vi "Create Value - Known Type.vi"(5 "JSON Compatible Type":T1=enum."Unknown", 7 "JSON Type":T2=enum."Unknown", 8 "error in (no error)":errorcluster, 10 "Value":variant) -> (0 "error out":errorcluster, 3 "JSON Tree":variant)   [LabVIEW 2014, in "i3-json.lvlib"]
doc: "Creates a new JSON Object of the given type"
uses:
  i3-json.lvlib
  JSON Types/JSON Type.ctl
  JSON Types/JSON Compatible Type.ctl
  JSON Types/JSON Variant Attribute.ctl
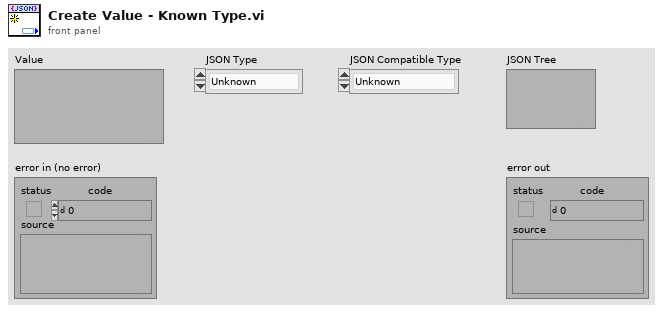
[diagram p1: front panel]
types:
  T1 = typedef "i3-json.lvlib/JSON Compatible Type.ctl" = enum16{"1D Double Array", "1D String Array", "1D Boolean Array", "Unknown"}
  T2 = typedef "i3-json.lvlib/JSON Type.ctl" = enum8{"JSON Compatible", "JSON Array", "JSON Object", "JSON Null", "Double", "String", "Boolean", "Unknown"}
  T3 = typedef "i3-json.lvlib/JSON Variant Attribute.ctl" = string
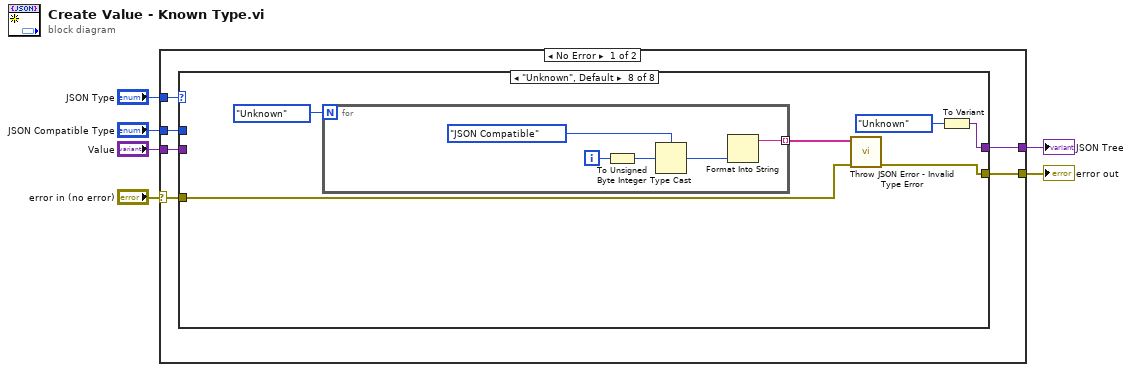
[diagram p0: block diagram]
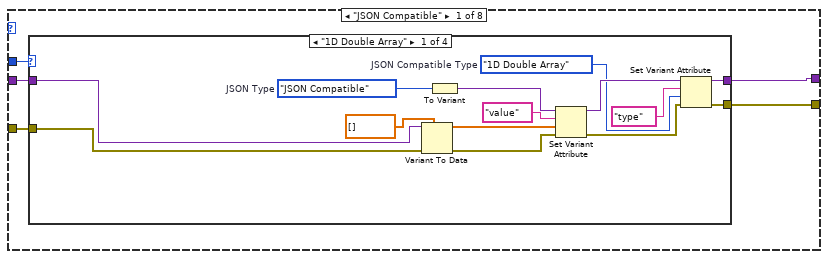
[diagram p2: hidden frame]
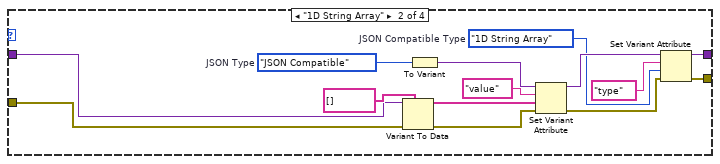
[diagram p3: hidden frame]
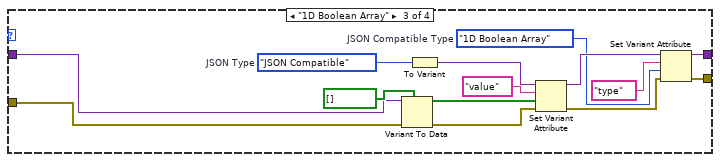
[diagram p4: hidden frame]
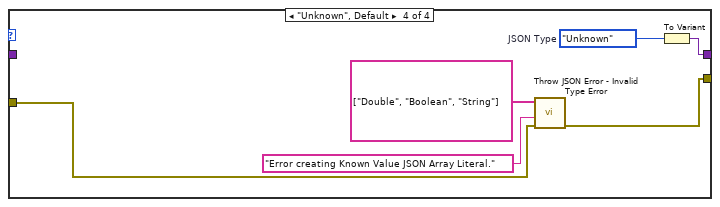
[diagram p5: hidden frame]
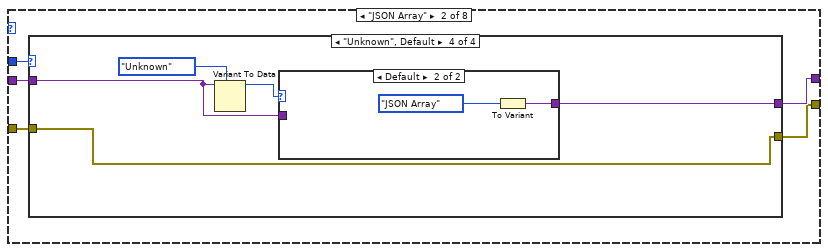
[diagram p6: hidden frame]
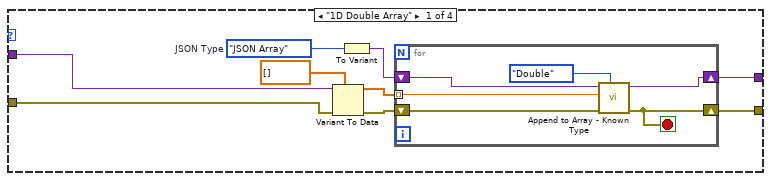
[diagram p7: hidden frame]
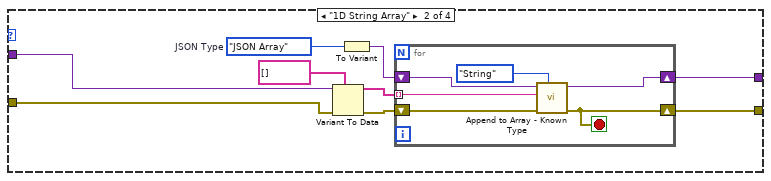
[diagram p8: hidden frame]
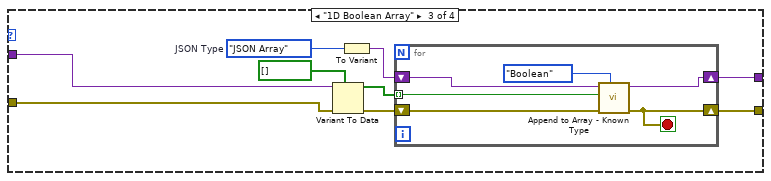
[diagram p9: hidden frame]
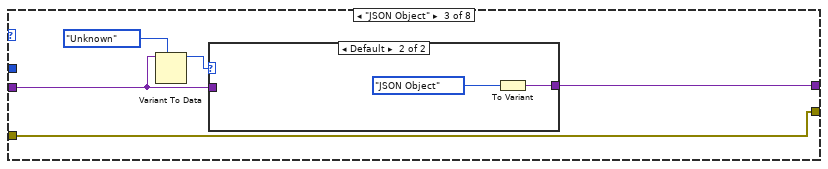
[diagram p11: hidden frame]
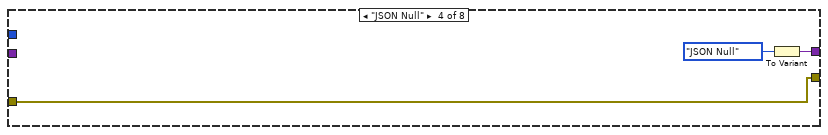
[diagram p13: hidden frame]
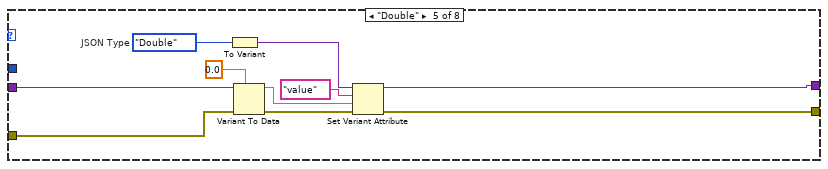
[diagram p14: hidden frame]
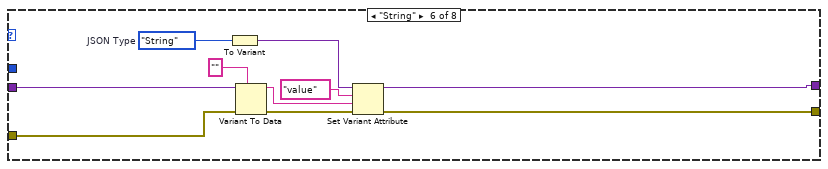
[diagram p15: hidden frame]
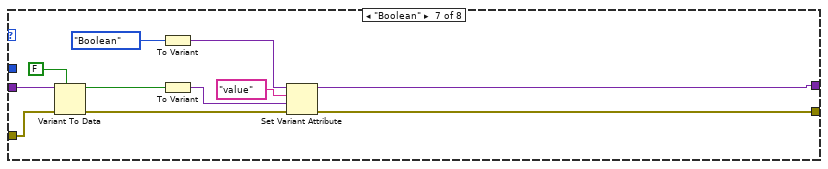
[diagram p16: hidden frame]
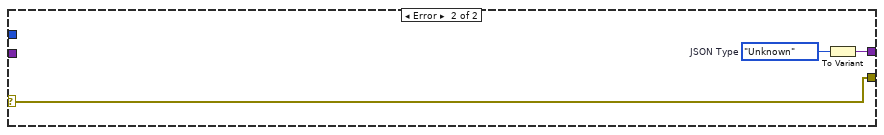
[diagram p17: hidden frame]
diagram:
  n1 = case shown="No Error" "error in (no error)" {
    selector: "error in (no error)" -> [w11 w177]
    tunnel: [w12 w177] -> w5
    tunnel: [w10 w178] -> w4
    tunnel: "JSON Type" -> [w9 _]
    tunnel: "JSON Compatible Type" -> [w8 _]
    tunnel: "Value" -> [w7 _]
    frame No Error {
      n2 = case shown="\"Unknown\", Default" w9 {
        tunnel: [w15 w66 w128 w132 w137 w147 w156 w168] -> w12
        tunnel: w11 -> [w14 w69 w128 w132 w143 w153 w163 w169]
        tunnel: [w16 w70 w125 w133 w135 w148 w157 w171] -> w10
        tunnel: w7 -> [w13 w67 w126 _ w142 w152 w164 _]
        tunnel: w8 -> [w17 w68 _ _ _ _ _ _]
        frame "JSON Compatible" {
          n3 = case shown="\"1D Double Array\"" w17 {
            tunnel: [w19 w38 w53 w64] -> w16
            tunnel: [w18 w37 w52 w60] -> w15
            tunnel: w14 -> [w22 w32 w47 w61]
            tunnel: w13 -> [w21 w35 w46 _]
            frame "1D Double Array" {
              w25 = JSON_Compatible_Type."1D Double Array"  # JSON Compatible Type
              w31 = JSON_Type."JSON Compatible"  # JSON Type
              n4 = Variant To Data(error in=w22, type=dbl[] [], Variant=w21) -> (data=w20:dbl[], error out=w23:errorcluster)
              n5 = To Variant(anything=w31) -> (Variant=w30:variant)
              n6 = Set Variant Attribute(Variant=w30, name=T3 "value" ("JSON Variant Attribute"), value=w20, error in=w23) -> (Variant out=w27:variant, error out=w29:errorcluster)  [unwired: 1 out]
              n7 = Set Variant Attribute(Variant=w27, name=T3 "type" ("JSON Variant Attribute"), value=w25, error in=w29) -> (Variant out=w19:variant, error out=w18:errorcluster)  [unwired: 1 out]
            }
            frame "1D String Array" {
              w39 = JSON_Compatible_Type."1D String Array"  # JSON Compatible Type
              w45 = JSON_Type."JSON Compatible"  # JSON Type
              n8 = Variant To Data(error in=w32, type=string[] [], Variant=w35) -> (data=w34:string[], error out=w33:errorcluster)
              n9 = To Variant(anything=w45) -> (Variant=w44:variant)
              n10 = Set Variant Attribute(Variant=w44, name=T3 "value" ("JSON Variant Attribute"), value=w34, error in=w33) -> (Variant out=w41:variant, error out=w43:errorcluster)  [unwired: 1 out]
              n11 = Set Variant Attribute(Variant=w41, name=T3 "type" ("JSON Variant Attribute"), value=w39, error in=w43) -> (Variant out=w38:variant, error out=w37:errorcluster)  [unwired: 1 out]
            }
            frame "1D Boolean Array" {
              w54 = JSON_Compatible_Type."1D Boolean Array"  # JSON Compatible Type
              w50 = JSON_Type."JSON Compatible"  # JSON Type
              n12 = Variant To Data(error in=w47, type=bool[] [], Variant=w46) -> (data=w49:bool[], error out=w48:errorcluster)
              n13 = To Variant(anything=w50) -> (Variant=w59:variant)
              n14 = Set Variant Attribute(Variant=w59, name=T3 "value" ("JSON Variant Attribute"), value=w49, error in=w48) -> (Variant out=w56:variant, error out=w58:errorcluster)  [unwired: 1 out]
              n15 = Set Variant Attribute(Variant=w56, name=T3 "type" ("JSON Variant Attribute"), value=w54, error in=w58) -> (Variant out=w53:variant, error out=w52:errorcluster)  [unwired: 1 out]
            }
            frame "Unknown", Default {
              w65 = JSON_Type."Unknown"  # JSON Type
              n16 = call "Throw JSON Error - Invalid Type Error.vi"("error in (no error)"=w61, "additional info"="Error creating Known Value JSON Array Literal.", "Valid Types"=string[] ["Double", "Boolean", "String"]) -> ("error out"=w60:errorcluster)  [unwired: 8 in]
              n17 = To Variant(anything=w65) -> (Variant=w64:variant)
            }
          }
        }
        frame "JSON Array" {
          n18 = case shown="\"Unknown\", Default" w68 {
            tunnel: [w71 w88 w104 w117] -> w70
            tunnel: w69 -> [w79 w87 w102 w118]
            tunnel: [w72 w89 w103 w118] -> w66
            tunnel: w67 -> [w76 w86 w101 w119]
            frame "1D Double Array" {
              w75 = JSON_Type."JSON Array"  # JSON Type
              n19 = Variant To Data(error in=w79, type=dbl[] [], Variant=w76) -> (data=w77:dbl[], error out=w73:errorcluster)
              n20 = To Variant(anything=w75) -> (Variant=w74:variant)
              n21 = for {
                shift-right: [w83] -> w71
                shift-left: w74 -> [w84]
                tunnel: w77 -> [w85] mode=indexing
                shift-right: [w80] -> w72
                shift-left: w73 -> [w81]
                stop <- w80 stop-if-true
                n22 = call "Append to Array - Known Type.vi"("JSON Type"=JSON_Type."Double", "error in (no error)"=w81, "Value"=w85, "JSON Tree in (JSON Array)"=w84) -> ("error out"=w80:errorcluster, "JSON Tree out (JSON Array)"=w83:variant)  [unwired: 6 in]
              }
            }
            frame "1D String Array" {
              w92 = JSON_Type."JSON Array"  # JSON Type
              n23 = Variant To Data(error in=w87, type=string[] [], Variant=w86) -> (data=w91:string[], error out=w94:errorcluster)
              n24 = To Variant(anything=w92) -> (Variant=w93:variant)
              n25 = for {
                shift-right: [w98] -> w88
                shift-left: w93 -> [w99]
                tunnel: w91 -> [w100] mode=indexing
                shift-right: [w95] -> w89
                shift-left: w94 -> [w96]
                stop <- w95 stop-if-true
                n26 = call "Append to Array - Known Type.vi"("JSON Type"=JSON_Type."String", "error in (no error)"=w96, "Value"=w100, "JSON Tree in (JSON Array)"=w99) -> ("error out"=w95:errorcluster, "JSON Tree out (JSON Array)"=w98:variant)  [unwired: 6 in]
              }
            }
            frame "1D Boolean Array" {
              w107 = JSON_Type."JSON Array"  # JSON Type
              n27 = Variant To Data(error in=w102, type=bool[] [], Variant=w101) -> (data=w106:bool[], error out=w109:errorcluster)
              n28 = To Variant(anything=w107) -> (Variant=w108:variant)
              n29 = for {
                shift-right: [w113] -> w104
                shift-left: w108 -> [w114]
                tunnel: w106 -> [w115] mode=indexing
                shift-right: [w110] -> w103
                shift-left: w109 -> [w111]
                stop <- w110 stop-if-true
                n30 = call "Append to Array - Known Type.vi"("JSON Type"=JSON_Type."Boolean", "error in (no error)"=w111, "Value"=w115, "JSON Tree in (JSON Array)"=w114) -> ("error out"=w110:errorcluster, "JSON Tree out (JSON Array)"=w113:variant)  [unwired: 6 in]
              }
            }
            frame "Unknown", Default {
              n31 = Variant To Data(type=JSON_Type."Unknown" ("JSON Type"), Variant=w119) -> (data=w116:T2)  [unwired: 1 in, 1 out]
              n32 = case shown="Default" w116 {
                tunnel: w119 -> [w121 _]
                tunnel: [w121 w122] -> w117
                frame "JSON Array" {
                }
                frame Default {
                  n33 = To Variant(anything=JSON_Type."JSON Array" ("JSON Type")) -> (Variant=w122:variant)
                }
              }
            }
          }
        }
        frame "JSON Object" {
          n34 = Variant To Data(type=JSON_Type."Unknown" ("JSON Type"), Variant=w126) -> (data=w124:T2)  [unwired: 1 in, 1 out]
          n35 = case shown="Default" w124 {
            tunnel: w126 -> [w129 _]
            tunnel: [w129 w130] -> w125
            frame "JSON Object" {
            }
            frame Default {
              n36 = To Variant(anything=JSON_Type."JSON Object" ("JSON Type")) -> (Variant=w130:variant)
            }
          }
        }
        frame "JSON Null" {
          n37 = To Variant(anything=JSON_Type."JSON Null" ("JSON Type")) -> (Variant=w133:variant)
        }
        frame "Double" {
          w141 = JSON_Type."Double"  # JSON Type
          n38 = To Variant(anything=w141) -> (Variant=w140:variant)
          n39 = Variant To Data(error in=w143, type=0.0 ("Numeric"), Variant=w142) -> (data=w136:dbl, error out=w138:errorcluster)
          n40 = Set Variant Attribute(Variant=w140, name=T3 "value" ("JSON Variant Attribute"), value=w136, error in=w138) -> (Variant out=w135:variant, error out=w137:errorcluster)  [unwired: 1 out]
        }
        frame "String" {
          w151 = JSON_Type."String"  # JSON Type
          n41 = To Variant(anything=w151) -> (Variant=w150:variant)
          n42 = Variant To Data(error in=w153, type="" ("String"), Variant=w152) -> (data=w145:string, error out=w146:errorcluster)
          n43 = Set Variant Attribute(Variant=w150, name=T3 "value" ("JSON Variant Attribute"), value=w145, error in=w146) -> (Variant out=w148:variant, error out=w147:errorcluster)  [unwired: 1 out]
        }
        frame "Boolean" {
          n44 = Variant To Data(error in=w163, type=FALSE ("data"), Variant=w164) -> (data=w158:bool, error out=w155:errorcluster)
          n45 = To Variant(anything=JSON_Type."Boolean" ("JSON Type")) -> (Variant=w161:variant)
          n46 = To Variant(anything=w158) -> (Variant=w159:variant)
          n47 = Set Variant Attribute(Variant=w161, name=T3 "value" ("JSON Variant Attribute"), value=w159, error in=w155) -> (Variant out=w157:variant, error out=w156:errorcluster)  [unwired: 1 out]
        }
        frame "Unknown", Default {
          n48 = for {
            N: JSON_Type."Unknown" ("JSON Type") -> [_]
            tunnel: [w176] -> w167 mode=indexing
            i -> [w173]
            n49 = To Unsigned Byte Integer(number=w173) -> (unsigned 8bit integer=w172:u8)
            n50 = Type Cast(type=JSON_Type."JSON Compatible" ("JSON Type"), x=w172) -> (*(type *) &x=w174:T2)
            n51 = Format Into String(w174) -> (resulting string=w176:string)  [unwired: 3 in, 1 out]
          }
          n52 = call "Throw JSON Error - Invalid Type Error.vi"("error in (no error)"=w169, "Valid Types"=w167) -> ("error out"=w168:errorcluster)  [unwired: 9 in]
          n53 = To Variant(anything=JSON_Type."Unknown" ("JSON Type")) -> (Variant=w171:variant)
        }
      }
    }
    frame Error {
      w179 = JSON_Type."Unknown"  # JSON Type
      n54 = To Variant(anything=w179) -> (Variant=w178:variant)
    }
  }
  "JSON Tree" <- w4
  "error out" <- w5
